vi "Pre Launch Init.vi"(11 "HamamatsuFluor in":refnum<class "HamamatsuFluor.lvclass">) -> (0 "error out":errorcluster, 3 "HamamatsuFluor out":refnum<class "HamamatsuFluor.lvclass">)   [LabVIEW 2020, in "DAQ Timed SPIM.lvlib" / "HamamatsuFluor_v2.lvlib" / "HamamatsuFluor.lvclass"]
doc: "(<B>Filename</B>: Actor Framework.lvlib:Actor.lvclass:Pre Launch Init.vi)\n\nDefines behavior that occurs after the Launch Nested Actor method is invoked but before the actor's Actor Core method begins running.\n\nBy default, this method does nothing. A descendant class may override it to define behavior."
uses:
  HamamatsuFluor.lvclass
  C:/WormSPIM/Labview/SPIM Engine/HW Timed SPIM/Abstract DAQ Triggered Actor/Abstract DAQ Triggered Actor.lvclass
  HamamatsuFluor.lvclass/HamamatsuFluor.ctl
  <vilib>/Utility/error.llb/Error Cluster From Error Code.vi
  Abstract DAQ Triggered Actor/Abstract DAQ Triggered Actor.lvclass
  <vilib>/ErrorRing/Error Ring.xnode
  WIN Memory Map.llb/WIN MMAP.lvlib
panel:
  in  "Default Save Path":path=path "E:/"
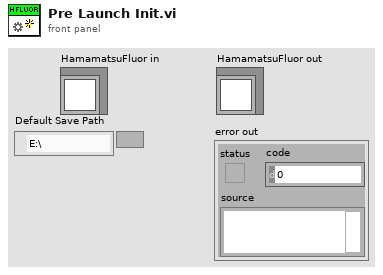
[diagram p1: front panel]
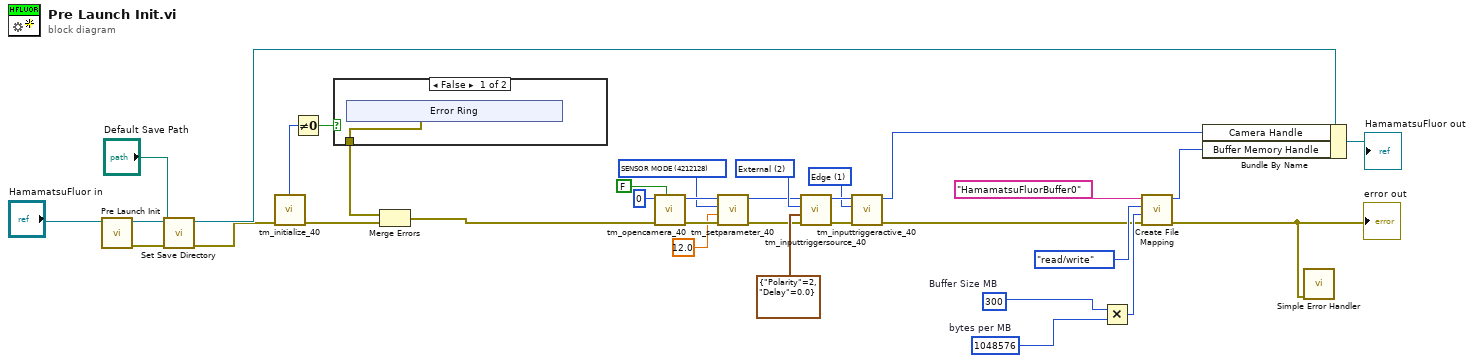
[diagram p0: block diagram]
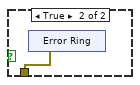
[diagram p2: hidden frame]
diagram:
  w14 = u32 300  # Buffer Size MB
  w16 = u32 1048576  # bytes per MB
  w26 = 1 items=["Edge"=1, "Level"=2, "Sync Readout"=3, "Point"=4] ("Active")
  w25 = 2 items=["Internal"=1, "External"=2, "Software"=3, "Master Pulse"=4] ("Source")
  w31 = u32 4212128 items=["SENSOR MODE"=4212128, "READOUT SPEED"=4211872, "READOUT DIRECTION"=4211904, "BIT PER CHANNEL"=4342976, "TRIGGER GLOBAL EXPOSURE"=2049680, "TRIGGER DELAY"=1066480, "INTERNAL TRIGGER HANDLING"=1066496, "SENSOR TEMPERATURE"=2115232, "SENSOR COOLER STATUS"=2115280, "EXPOSURE TIME"=2049184, "DEFECT CORRECT MODE"=4670368, "HOT PIXEL CORRECT LEVEL"=4670400, "BINNING"=4215968, "TIMING READOUT TIME"=4223904, "INTERNAL FRAME RATE"=4225952, "INTERNAL FRAME INTERVAL"=4225968, "INTERNAL LINE SPEED"=4226000, "INTERNAL LINE INTERVAL"=4226016, "IMAGE WIDTH"=4343200, "IMAGE HEIGHT"=4343216, "IMAGE ROWBYTES"=4343232, "IMAGE FRAMEBYTES"=4343248, "IMAGE PIXEL TYPE"=4343296, "NUMBER OF OUTPUT TRIGGER CONNECTOR"=1852320, "OUTPUT TRIGGER SOURCE[0]"=1852576, "OUTPUT TRIGGER SOURCE[1]"=1852832, "OUTPUT TRIGGER SOURCE[2]"=1853088, "OUTPUT TRIGGER POLARITY[0]"=1852592, "OUTPUT TRIGGER POLARITY[1]"=1852848, "OUTPUT TRIGGER POLARITY[2]"=1853104, "OUTPUT TRIGGER ACTIVE[0]"=1852608, "OUTPUT TRIGGER ACTIVE[1]"=1852864, "OUTPUT TRIGGER ACTIVE[2]"=1853120, "OUTPUT TRIGGER DELAY[0]"=1852624, "OUTPUT TRIGGER DELAY[1]"=1852880, "OUTPUT TRIGGER DELAY[2]"=1853136, "OUTPUT TRIGGER PERIOD[0]"=1852640, "OUTPUT TRIGGER PERIOD[1]"=1852896, "OUTPUT TRIGGER PERIOD[2]"=1853152, "OUTPUT TRIGGER KIND[0]"=1852656, "OUTPUT TRIGGER KIND[1]"=1852912, "OUTPUT TRIGGER KIND[2]"=1853168, "OUTPUT TRIGGER BASE SENSOR[0]"=1852672, "OUTPUT TRIGGER BASE SENSOR[1]"=1852928, "OUTPUT TRIGGER BASE SENSOR[2]"=1853184, "OUTPUT TRIGGER PRE HSYNC COUNT"=1852704] ("Parameter")
  n1 = call-parent "Pre Launch Init.vi"("Actor in"="HamamatsuFluor in") -> ("error out"=w20:errorcluster, "Actor out"=w19:refnum<class "HamamatsuFluor.lvclass">)  [unwired: 9 in]
  n2 = call "Set Save Directory.vi"("error in (no error)"=w20, "Path"="Default Save Path", "Abstract DAQ Triggered Actor in"=w19) -> ("error out"=w6:errorcluster, "Abstract DAQ Triggered Actor out"=w10:refnum<class "HamamatsuFluor.lvclass">)  [unwired: 7 in]
  n3 = call <userlib>:"tm_initialize_40.vi"("error in (no error)"=w6) -> ("error out"=w2:errorcluster, "Number Of Cameras"=w5:u32)  [unwired: 7 in, 2 out]
  n4 = Not Equal To 0?(x=w5) -> (x != 0?=w4:bool)
  n5 = case shown="False" w4 {
    tunnel: [w35 w40] -> w3
    frame False {
      n6 = xnode "Error Ring"() -> ("error out"=w35:errorcluster)
    }
    frame True {
      n7 = xnode "Error Ring"() -> ("error out"=w40:errorcluster)
    }
  }
  n8 = Merge Errors(w3, w2) -> (w1:errorcluster)
  n9 = call <userlib>:"tm_opencamera_40.vi"("Force Open"=FALSE, "error in (no error)"=w1, "Camera Index"=u32 0) -> ("error out"=w32:errorcluster, "Handle out"=w33:u32)  [unwired: 6 in, 1 out]
  n10 = call <userlib>:"tm_setparameter_40.vi"("error in (no error)"=w32, "Value in"=12.0, "Parameter"=w31, "Handle in"=w33) -> ("error out"=w23:errorcluster, "Handle out"=w22:u32)  [unwired: 6 in]
  n11 = call <userlib>:"tm_inputtriggersource_40.vi"("error in (no error)"=w23, "External Options"=cluster{"Polarity":i32, "Delay":dbl} {"Polarity"=2, "Delay"=0.0}, "Source"=w25, "Handle in"=w22) -> ("error out"=w27:errorcluster, "Handle out"=w28:u32)  [unwired: 6 in]
  n12 = call <userlib>:"tm_inputtriggeractive_40.vi"("error in (no error)"=w27, "Active"=w26, "Handle in"=w28) -> ("error out"=w9:errorcluster, "Handle out"=w21:u32)  [unwired: 7 in]
  n13 = Multiply(x=w14, y=w16) -> (x*y=w13:u32)
  n14 = call "Create File Mapping.vi"("error in (no error)"=w9, "map size"=w13, "access (0:read/write)"=enum16{"read/write", "read-only", "write-only"}."read/write", "map file name"="HamamatsuFluorBuffer0") -> ("error out"=w8:errorcluster, "handle"=w7:u64)  [unwired: 6 in]
  "error out" <- w8
  n15 = Bundle By Name(cluster=w10, "Camera Handle"=w21, "Buffer Memory Handle"=w7) -> (→"HamamatsuFluor out":refnum<class "HamamatsuFluor.lvclass">)
  n16 = call <vilib>:"Simple Error Handler.vi"("error in (no error)"=w8) -> ()  [unwired: 4 in, 5 out]
